vi "GDSString_AttributeTextToAttributeType.vi"(6 "Classes":T1[](array[typedef]), 7 "RemoveAttributesWithEmptynames(False)":bool, 9 "MethodText":string, 10 "DefaultAccessScope(Private)":T2=enum."private", 11 "Attribute,Struct,Enum-Text":string) -> (0 "ClassesOrTypesDependency":string[](array[string]), 1 "Structs":T3[](array[typedef]), 2 "Enums":T7[](array[typedef]), 3 "Attributes":T5[](array[typedef]))   [LabVIEW 2020]
uses:
  CommonVIs/CommonVIs_AttributeType.ctl
  CommonVIs/CommonVIs_AttributeDataType.ctl
  GDSString_AccessScopeModifierType.ctl
  CommonVIs/CommonVIs_EnumType.ctl
  GDSString_ModifierType.ctl
  CommonVIs/CommonVIs_StructType.ctl
  CommonVIs/CommonVIs_ClassNamePathType.ctl
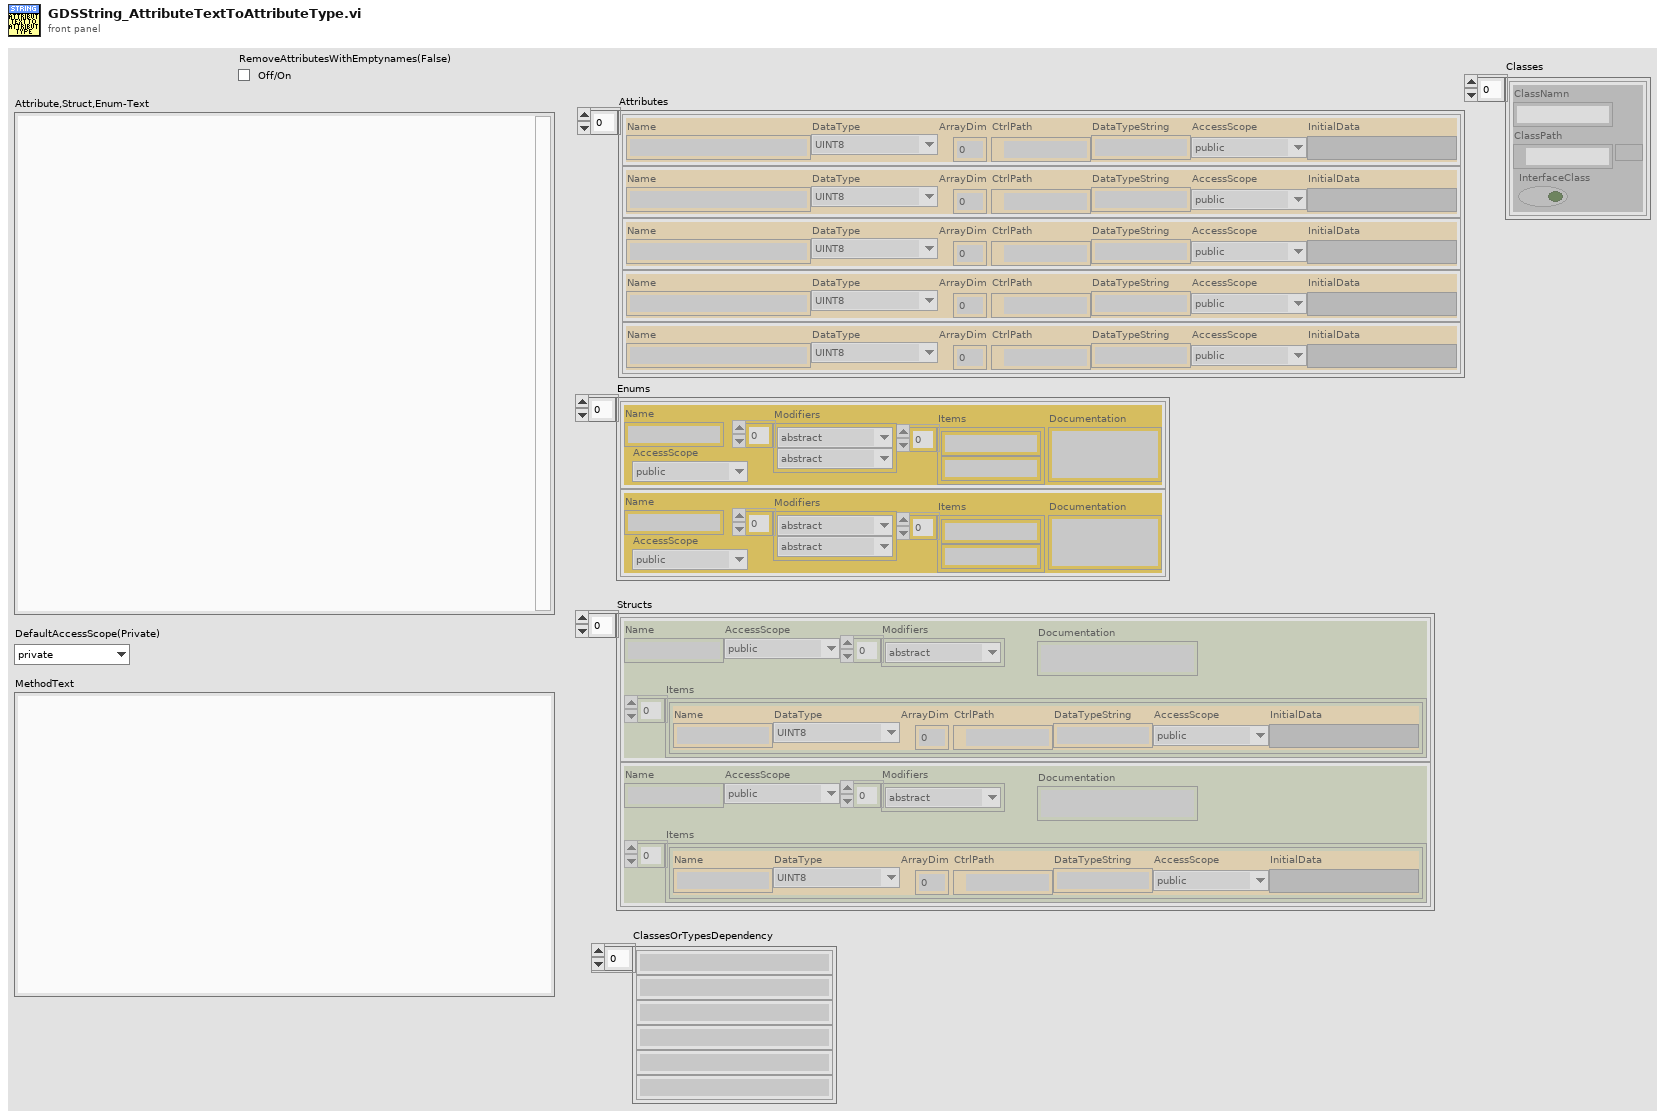
[diagram p1: front panel]
types:
  T1 = typedef "CommonVIs_ClassNamePathType.ctl" = cluster{"ClassNamn":string, "ClassPath":path, "InterfaceClass":bool}
  T2 = typedef "GDSString_AccessScopeModifierType.ctl" = enum16{"public", "private", "protected", "internal"}
  T3 = typedef "CommonVIs_StructType.ctl" = cluster{"Name":string, "AccessScope":T2, "Modifiers":T4[], "Items":T5[], "Documentation":string}
  T4 = typedef "GDSString_ModifierType.ctl" = enum16{"abstract", "static", "final", "synchronized", "strictfp", "async", "const", "event", "extern", "new", "native ", "override", "partial", "readonly", "sealed", "unsafe", "virtual", "volatile"}
  T5 = typedef "CommonVIs_AttributeType.ctl" = cluster{"Name":string, "DataType":T6, "ArrayDim":i32, "CtrlPath":path, "DataTypeString":string, "AccessScope":T2, "InitialData":variant}
  T6 = typedef "CommonVIs_AttributeDataType.ctl" = enum16{"UINT8", "INT8", "UINT16", "INT16", "UINT32", "INT32", "UINT64", "INT64", "SGL", "DBL", "EXT", "CSG", "CDB", "CXT", "TimeStamp", "STRING", "PATH", "BOOL", "ENUM", "RefNum", "VIRefNum", "LabVIEW Class", "Cluster", "Variant", "TypeDef", "Waveform", "LabVIEW Object", "Other", "void", "Set", "Map"}
  T7 = typedef "CommonVIs_EnumType.ctl" = cluster{"Name":string, "AccessScope":T2, "Modifiers":T4[], "Items":string[], "Documentation":string}
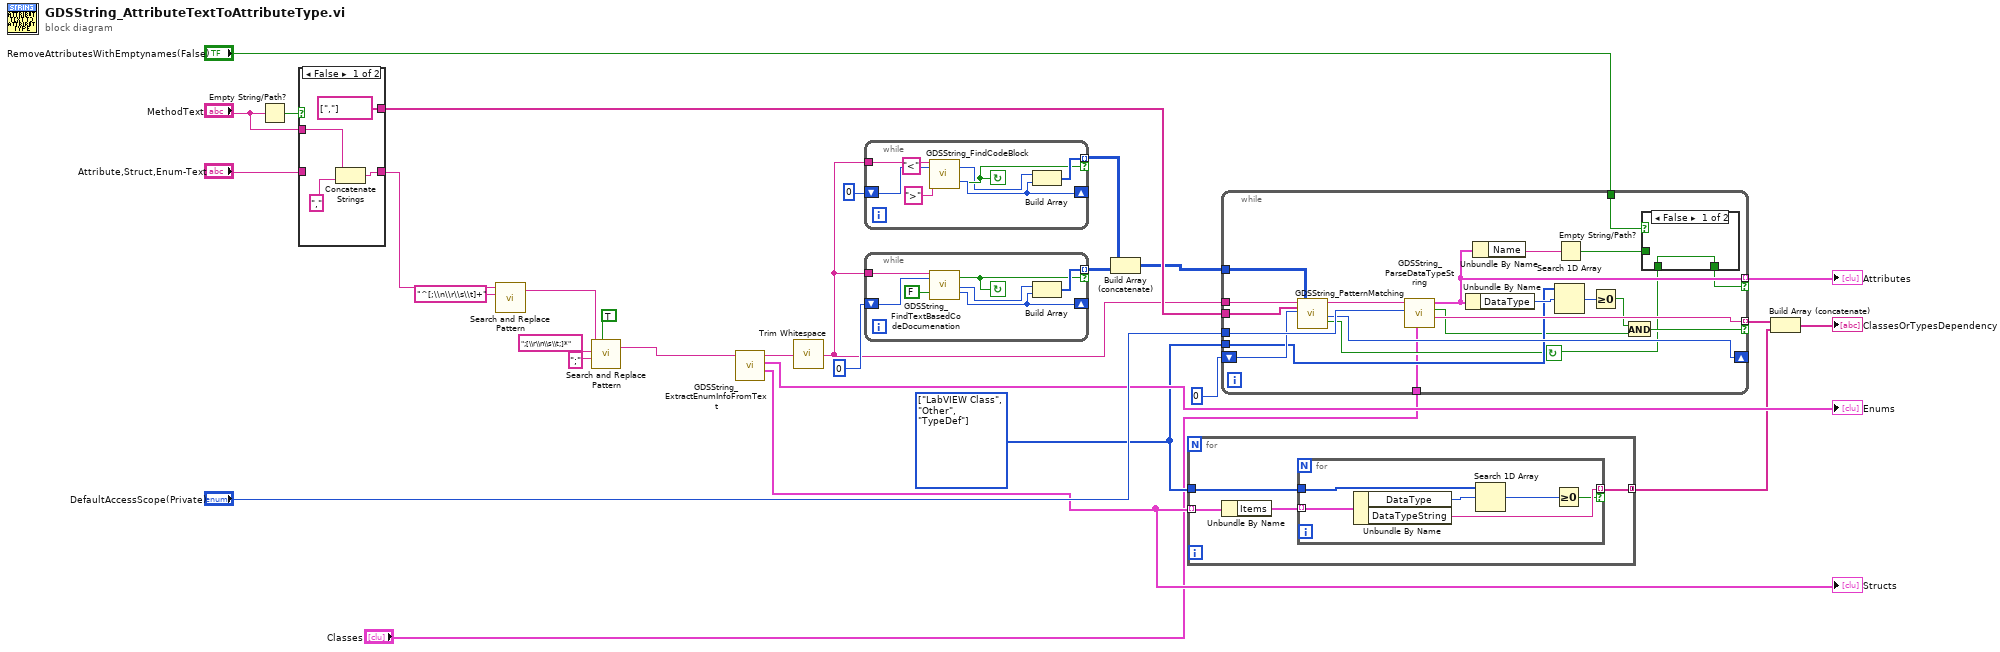
[diagram p0: block diagram]
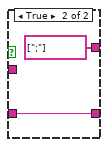
[diagram p2: hidden frame]
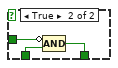
[diagram p3: hidden frame]
diagram:
  w19 = T6[] [enum."LabVIEW Class", enum."Other", enum."TypeDef"] items=["UINT8", "INT8", "UINT16", "INT16", "UINT32", "INT32", "UINT64", "INT64", "SGL", "DBL", "EXT", "CSG", "CDB", "CXT", "TimeStamp", "STRING", "PATH", "BOOL", "ENUM", "RefNum", "VIRefNum", "LabVIEW Class", "Cluster", "Variant", "TypeDef", "Waveform", "LabVIEW Object", "Other", "void", "Set", "Map"] ("1D array")
  n1 = Empty String/Path?(string/path="MethodText") -> (empty?=w16:bool)
  n2 = case shown="False" w16 {
    tunnel: [string[] [","] ("PatternMatchingStrings") string[] [";"] ("PatternMatchingStrings")] -> w24
    tunnel: "MethodText" -> [w32 _]
    tunnel: [w31 w34] -> w8
    tunnel: "Attribute,Struct,Enum-Text" -> [_ w34]
    frame False {
      n3 = Concatenate Strings(w32, "," ("regular expression")) -> (w31:string)
    }
    frame True {
    }
  }
  n4 = call <vilib>:"Search and Replace Pattern.vi"("string"=w8, "regular expression (\"\")"="^[;\\n\\r\\s\\t]+" ("regular expression (\"\")")) -> ("result string"=w7:string)  [unwired: 3 in, 1 out]
  n5 = call <vilib>:"Search and Replace Pattern.vi"("string"=w7, "regular expression (\"\")"=";[\\r\\n\\s\\t;]*" ("string"), "replace string (\"\")"=";" ("regular expression (\"\")"), "replace all? (F)"=TRUE) -> ("result string"=w6:string)  [unwired: 1 in, 1 out]
  n6 = call "GDSString_ExtractEnumInfoFromText.vi"("AttributeStringIn"=w6) -> ("Structs"=w20:T3[], "Enums"=→"Enums":T7[], "StructsAndEnumsRemoved"=w23:string)  [unwired: 7 in, 1 out]
  "Structs" <- w20
  n7 = call <vilib>:"Trim Whitespace.vi"("string"=w23) -> ("trimmed string"=w12:string)  [unwired: 1 in]
  n8 = while {
    tunnel: w12 -> [w43]
    shift-right: [w42] -> _
    shift-left: 0 ("offset past match") -> [w41]
    tunnel: [w40] -> w10 mode=indexing if=w39
    stop <- w39 continue-if-true
    n9 = call "GDSString_FindCodeBlock.vi"("Text"=w43, "StringStartOffset(Default=-1 => 0 for Forward, StrLenght for Backwards)"=w41, "CodeBlockStartCharacter( { )"="<", "CodeBlockEndCharacter( } )"=">") -> ("found"=w39:bool, "BlockStart(Outside)"=w36:i32, "BlockEnd(Outside)"=w42:i32)  [unwired: 7 in, 6 out]
    n10 = Build Array(w36, w42) -> (w40:i32[])
  }
  n11 = while {
    tunnel: w12 -> [w50]
    shift-right: [w48] -> _
    shift-left: 0 ("offset past match") -> [w47]
    tunnel: [w46] -> w21 mode=indexing if=w45
    stop <- w45 continue-if-true
    n12 = call "GDSString_FindTextBasedCodeDocumenation.vi"("Text"=w50, "StringStartOffset(Default=-1 => 0 for Forward, StrLenght for Backwards)"=w47, "CommentHasToBeTheFirstItem(True)"=FALSE) -> ("Found"=w45:bool, "IndexBeforeDocument(Or after when searching Backwards)"=w49:i32, "IndexAfterDocument(Or before when searching Backwards)"=w48:i32)  [unwired: 12 in, 2 out]
    n13 = Build Array(w49, w48) -> (w46:i32[])
  }
  n14 = Build Array (concatenate)(w10, w21) -> (w11:i32[][])
  n15 = for {
    tunnel: w20 -> [w54] mode=indexing
    tunnel: w19 -> [w52]
    tunnel: [w51] -> w18 mode=concatenating
    n16 = Unbundle By Name(w54) -> ("Items"=w53:T5[])
    n17 = for {
      tunnel: w53 -> [w60] mode=indexing
      tunnel: w52 -> [w57]
      tunnel: [w56] -> w51 mode=indexing if=w55
      n18 = Unbundle By Name(w60) -> ("DataType"=w58:T6, "DataTypeString"=w56:string)
      n19 = Search 1D Array(1D array=w57, element=w58) -> (index of element=w59:i32)  [unwired: 1 in]
      n20 = Greater Or Equal To 0?(x=w59) -> (x >= 0?=w55:bool)
    }
  }
  n21 = while {
    tunnel: [w67] -> w29 mode=indexing if=w63
    tunnel: "DefaultAccessScope(Private)" -> [w80]
    tunnel: [w79] -> w28 mode=indexing if=w76
    tunnel: w24 -> [w74]
    tunnel: w12 -> [w73]
    shift-right: [w71] -> _
    shift-left: 0 ("offset past match") -> [w72]
    tunnel: w11 -> [w69]
    tunnel: w19 -> [w70]
    tunnel: "RemoveAttributesWithEmptynames(False)" -> [w62]
    tunnel: "Classes" -> [w61]
    stop <- w64 continue-if-true
    n22 = call "GDSString_PatternMatching.vi"("TextIn"=w73, "PatternMatchingStrings"=w74, "StringStartOffset(Default=-1 => 0 for Forward, StrLenght for Backwards)"=w72, "IgnoreMatchesWithinThesePositions"=w69) -> ("TextBefore"=w81:string, "IndexAfterMatch(Or before when searching Backwards)"=w71:i32, "Found"=w64:bool)  [unwired: 9 in, 4 out]
    n23 = call "GDSString_ParseDataTypeString.vi"("Classes"=w61, "DefaultAccessScope(Private)"=w80, "InputText"=w81) -> ("DataTypeString"=w79:string, "Found"=w68:bool, "DataType"=w67:T5)  [unwired: 6 in]
    n24 = Unbundle By Name(w67) -> ("DataType"=w75:T6)
    n25 = Unbundle By Name(w67) -> ("Name"=w66:string)
    n26 = Search 1D Array(1D array=w70, element=w75) -> (index of element=w78:i32)  [unwired: 1 in]
    n27 = Empty String/Path?(string/path=w66) -> (empty?=w65:bool)
    n28 = Greater Or Equal To 0?(x=w78) -> (x >= 0?=w77:bool)
    n29 = And(x=w77, y=w68) -> (x .and. y?=w76:bool)
    n30 = case shown="False" w62 {
      tunnel: w65 -> [_ w85]
      tunnel: w64 -> [w82 w84]
      tunnel: [w82 w83] -> w63
      frame False {
      }
      frame True {
        n31 = Compound Arithmetic op=AND(invert w85, w84) -> (w83:bool)
      }
    }
  }
  "Attributes" <- w29
  n32 = Build Array (concatenate)(w28, w18) -> (→"ClassesOrTypesDependency":string[])
